vi "DriverStation Wait for Update.vi"(11 "DS occurrence":refnum<k4>) -> (3 "mode":u64)   [LabVIEW 2023]
uses:
  <vilib>/MRC/MrcLib.lvlib
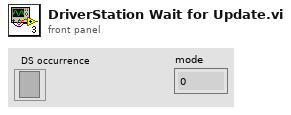
[diagram p1: front panel]
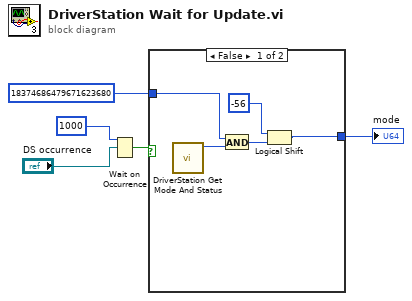
[diagram p0: block diagram]
diagram:
  n1 = Wait on Occurrence(2:"DS occurrence", 3:1000 ("ms timeout (-1)")) -> (0:w3:bool)  [unwired: 1 in]
  n2 = case shown="False" w3 {
    tunnel: u64 18374686479671623680 ("x") -> [w9 _]
    tunnel: [w6 _] -> w1
    frame False {
      n3 = call <vilib>:"DriverStation Get Mode And Status.vi"() -> ("currentOpMode"=w10:u64)  [unwired: 6 in, 5 out]
      n4 = And(x=w9, y=w10) -> (x .and. y?=w8:u64)
      n5 = Logical Shift(y=i16 -56, x=w8) -> (x << y=w6:u64)
    }
    frame True {
    }
  }
  "mode" <- w1
